vi "Merge Task Rows.vi"(8 "error in":errorcluster, 10 "Changes":T1[](array[typedef]), 11 "Task Rows in":T1[](array[typedef])) -> (0 "error out":errorcluster, 3 "Task Rows out":T1[](array[typedef]))   [LabVIEW 2026]
doc: "Merges Changes into a list of Task Edit Row clusters {Task Name, Active}, matching by exact Task Name: a row whose name is already in the list replaces that entry (so its Active wins); a new name is appended at the end; a row with an empty name is skipped. Rows are applied in order, so a later row for the same name wins. Nothing is removed and nothing is written - New Project.vi uses it to keep its full task list in step with the Tasks control.\n\nInputs: Task Rows in; Changes; error in.\nOutputs: Task Rows out; error out (error in passed through).\n\nGenerated by: Claude"
uses:
  Task Edit Row.ctl
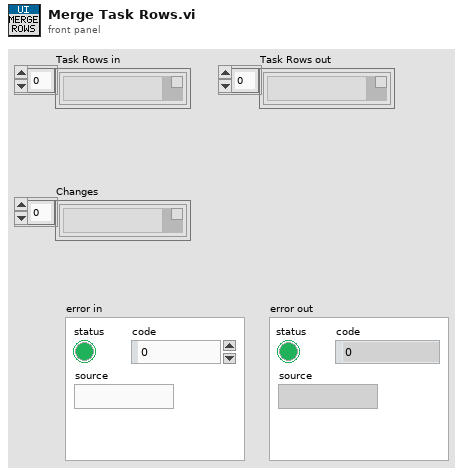
[diagram p1: front panel]
types:
  T1 = typedef "Task Edit Row.ctl" = cluster{"Task Name":string, "Active":bool}
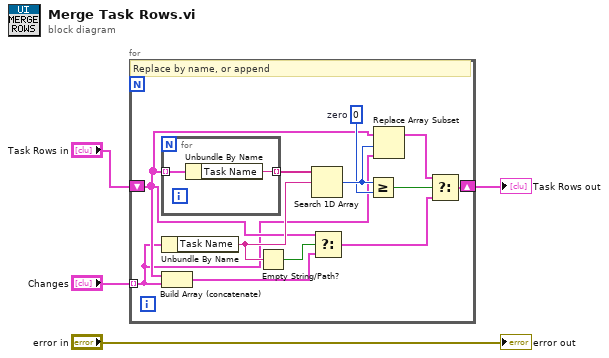
[diagram p0: block diagram]
diagram:
  n1 = for {
    tunnel: "Changes" -> [w5] mode=indexing
    shift-right: [w7] -> w4
    shift-left: "Task Rows in" -> [w6]
    w8 = 0  # zero
    # "Replace by name, or append"
    n2 = for {
      tunnel: w6 -> [w17] mode=indexing
      tunnel: [w18] -> w9 mode=indexing
      n3 = Unbundle By Name(w17) -> ("Task Name"=w18:string)
    }
    n4 = Unbundle By Name(w5) -> ("Task Name"=w10:string)
    n5 = Build Array (concatenate)(w6, w5) -> (w15:T1[])
    n6 = Empty String/Path?(string/path=w10) -> (empty?=w13:bool)
    n7 = Search 1D Array(1D array=w9, element=w10) -> (index of element=w11:i32)  [unwired: 1 in]
    n8 = Select(t=w6, s=w13, f=w15) -> (s? t:f=w16:T1[])
    n9 = Greater Or Equal?(x=w11, y=w8) -> (x >= y?=w12:bool)
    n10 = Replace Array Subset(array=w6, new element=w5, index=w11) -> (w14:T1[])
    n11 = Select(t=w14, s=w12, f=w16) -> (s? t:f=w7:T1[])
  }
  "Task Rows out" <- w4
  "error out" <- "error in"
